vi "OnConnectionEvent_Request.vi"(4 "Connection":refnum<vi>, 5 "事件数据":T1, 6 "控件引用":refnum<k24>, 7 "事件通用数据":cluster{"事件源":i32, "事件类型":u32, "时间标识":u32}) -> ()   [LabVIEW 2018]
uses:
  C:/users data/project/MES/MES v4.5 20250917/module/CFX/CFX_dll/CFX.dll
  CFX_dll/CFX.dll
panel:
  out "ConnectionEstablished":i32(ring) items=["ConnectionEstablished", "ConnectionFailed", "ConnectionInterrupted", "ConnectionClosed"]
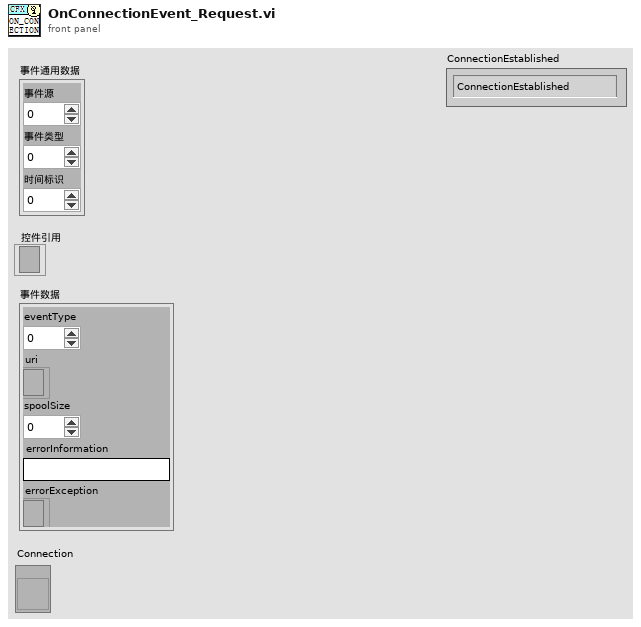
[diagram p1: front panel]
types:
  T1 = cluster{"eventType":i32, "uri":refnum<k24>, "spoolSize":i32, "errorInformation":string, "errorException":refnum<k24>}
  T2 = cluster{"ConnectionEstablished":i32, "ConnectionLog":string}
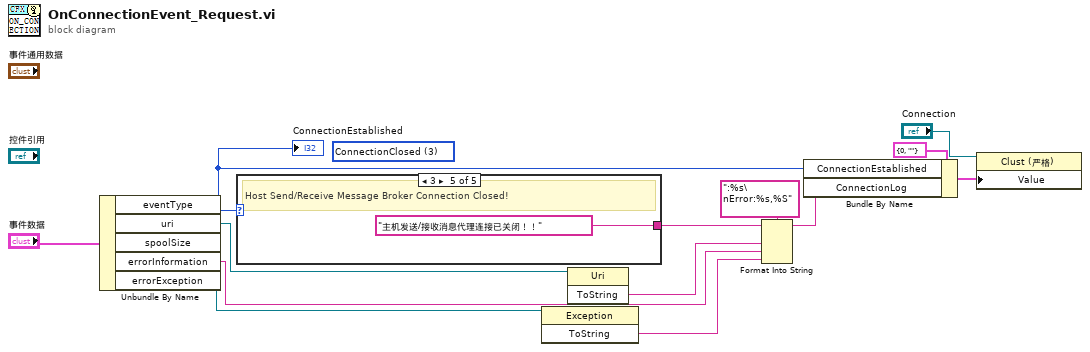
[diagram p0: block diagram]
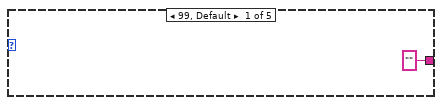
[diagram p2: hidden frame]
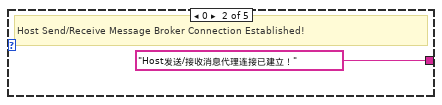
[diagram p3: hidden frame]
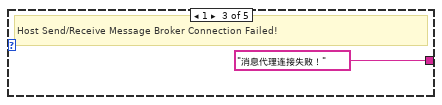
[diagram p4: hidden frame]
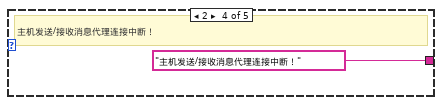
[diagram p5: hidden frame]
diagram:
  (unwired) 3 items=["ConnectionEstablished", "ConnectionFailed", "ConnectionInterrupted", "ConnectionClosed"] ("ConnectionEstablished")
  n1 = Unbundle By Name("事件数据") -> ("eventType"=w9:i32, "uri"=w7:refnum<k24>, "errorInformation"=w3:string, "errorException"=w2:refnum<k24>)  [unwired: 1 out]
  "ConnectionEstablished" <- w9
  n2 = case shown="3" w9 {
    tunnel: ["" ("ConnectionLog") "Host发送/接收消息代理连接已建立！" ("ConnectionLog") "消息代理连接失败！" ("ConnectionLog") "主机发送/接收消息代理连接中断！" ("ConnectionLog") "主机发送/接收消息代理连接已关闭！！" ("ConnectionLog")] -> w8
    frame 99, Default {
    }
    frame 0 {
      # "Host Send/Receive Message Broker Connection Established!"
    }
    frame 1 {
      # "Host Send/Receive Message Broker Connection Failed!"
    }
    frame 2 {
      # "主机发送/接收消息代理连接中断！"
    }
    frame 3 {
      # "Host Send/Receive Message Broker Connection Closed!"
    }
  }
  n3 = invoke class="Exception" method="ToString"(reference=w2) -> ("ToString"=w1:string)  [unwired: 2 in, 2 out]
  n4 = invoke class="Uri" method="ToString"(reference=w7) -> ("ToString"=w4:string)  [unwired: 2 in, 2 out]
  n5 = Format Into String(format string=":%s\nError:%s,%S" ("格式字符串"), initial string=w8, w4, w3, w1) -> (resulting string=w6:string)  [unwired: 1 in, 1 out]
  n6 = Bundle By Name(cluster=T2 {"ConnectionEstablished"=0, "ConnectionLog"=""} ("值"), "ConnectionEstablished"=w9, "ConnectionLog"=w6) -> (w10:T2)
  n7 = property class="Clust (严格)"(reference="Connection", "Value"=w10) -> ()  [unwired: 1 in, 2 out]
